vi "OwnCompat20261012_Native_GetWhileInfo_v3.vi"() -> ()   [LabVIEW 2024]
panel:
  out "error out":errorcluster caption="错误输出"
  out "counter_id":u32
  in  "counter_id type":u32
  out "stop_id":u32
  in  "stop_id type":u32
  out "diagram_id":u32
  in  "diagram_id type":u32
  in  "loop_id":u32
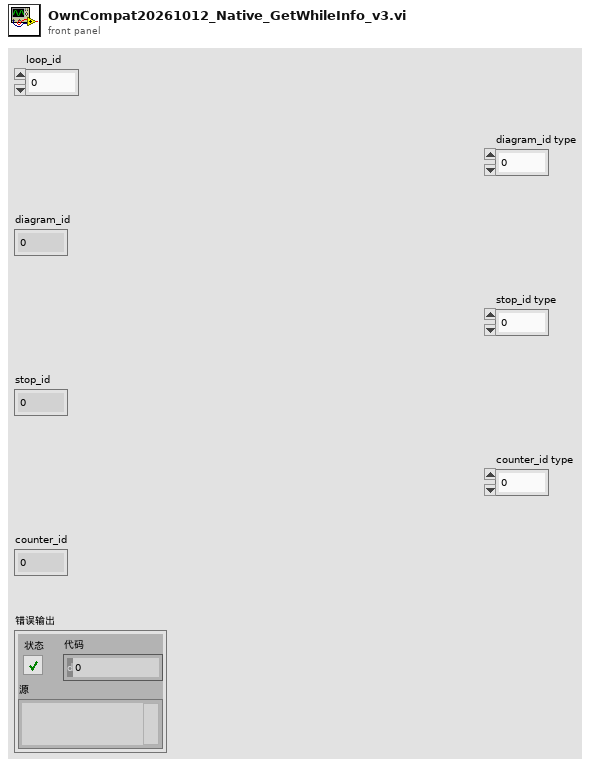
[diagram p1: front panel]
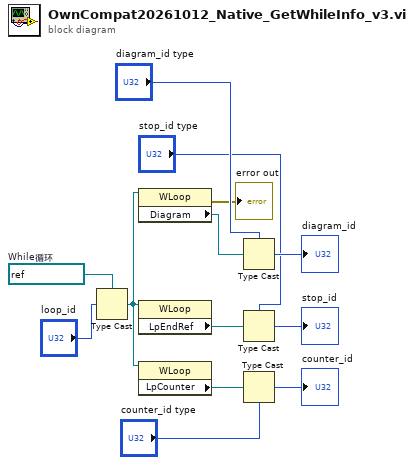
[diagram p0: block diagram]
diagram:
  w12 = refnum<vi> refnum  # While循环
  n1 = Type Cast ("强制类型转换")(type=w12, x="loop_id") -> (*(type *) &x=w11:refnum<vi>)
  n2 = property on="属性节点" class="WLoop"(reference=w11) -> (error out=→"error out":errorcluster, "Diagram"=w10:refnum<vi>)  [unwired: 1 in, 1 out]
  n3 = property on="属性节点" class="WLoop"(reference=w11) -> ("LpEndRef"=w7:refnum<vi>)  [unwired: 1 in, 2 out]
  n4 = property on="属性节点" class="WLoop"(reference=w11) -> ("LpCounter"=w4:refnum<vi>)  [unwired: 1 in, 2 out]
  n5 = Type Cast ("强制类型转换")(type="diagram_id type", x=w10) -> (*(type *) &x=→"diagram_id":u32)
  n6 = Type Cast ("强制类型转换")(type="stop_id type", x=w7) -> (*(type *) &x=→"stop_id":u32)
  n7 = Type Cast ("强制类型转换")(type="counter_id type", x=w4) -> (*(type *) &x=→"counter_id":u32)
